vi "LinearSystemSim_Update.vi"(6 "dT_Seconds":dbl=0.02, 11 "in LinearSystemSim":T1) -> (0 "Error":bool, 3 "out LinearSystemSim":T1)   [LabVIEW 2019, in "Trajectory_Library.lvlib"]
doc: "Updates the simulation.\n \nInputs:\n - LinearSystemSim -- Data cluster\n - dtSeconds -- The time between updates.\n\nOutputs:\n - OutLinearSystemSim -- Updated data cluster\n - Error -- If TRUE, an error occured."
uses:
  Trajectory_Library.lvlib
  TypeDef/LINEAR_SYSTEM_SIM.ctl
  TypeDef/LINEAR_SYSTEM.ctl
  <vilib>/Analysis/Matrix/Datatypes/RealMatrix.ctl
  <vilib>/Analysis/Matrix/NI_Matrix.lvlib
panel:
  # "<States, 1>"
  # "<Outputs, 1>"
  # "<Inputs, 1>"
  # "<Outputs, 1>"
  # "<States,States>"
  # "<States,Inputs>"
  # "<Outputs,States>"
  # "<Outputs,Inputs>"
  # "<States, 1>"
  # "<Outputs, 1>"
  # "<Inputs, 1>"
  # "<Outputs, 1>"
  # "<States,States>"
  # "<States,Inputs>"
  # "<Outputs,States>"
  # "<Outputs,Inputs>"
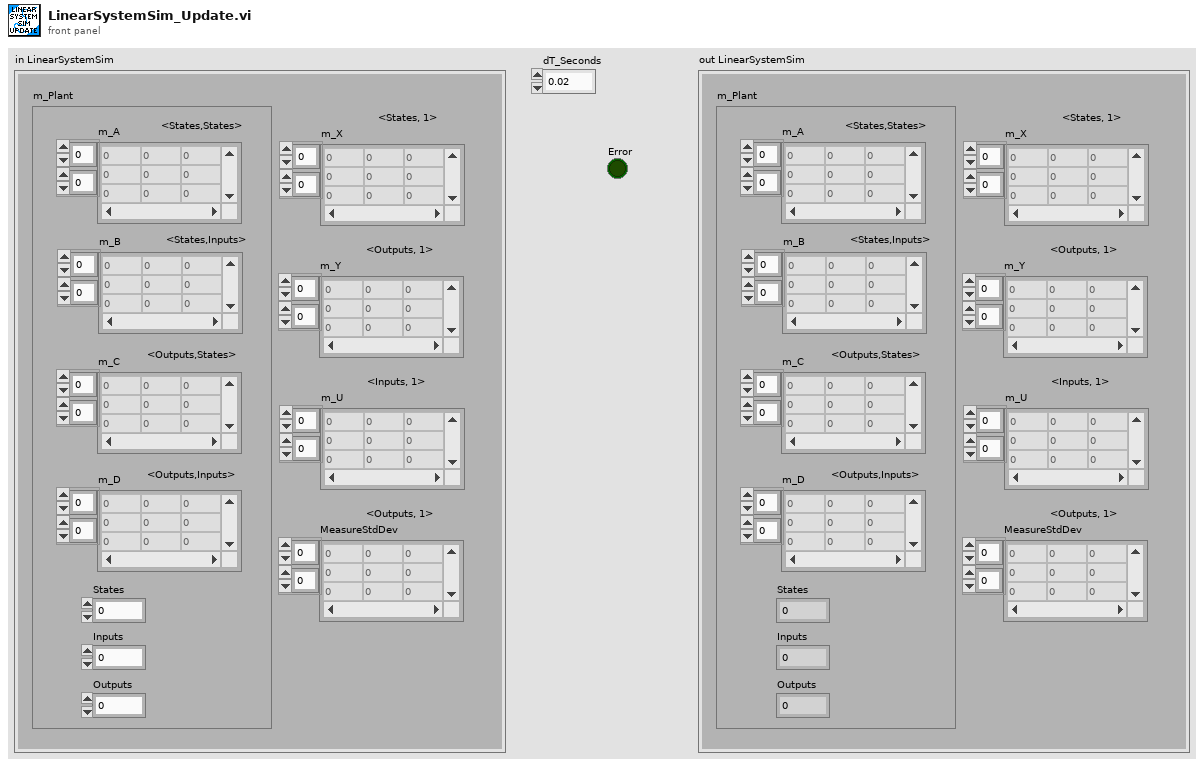
[diagram p1: front panel]
types:
  T1 = typedef "Trajectory_Library.lvlib/LINEAR_SYSTEM_SIM.ctl" = cluster{"m_Plant":T2, "m_X":T3, "m_Y":T3, "m_U":T3, "MeasureStdDev":T3}
  T2 = typedef "Trajectory_Library.lvlib/LINEAR_SYSTEM.ctl" = cluster{"m_A":T3, "m_B":T3, "m_C":T3, "m_D":T3, "States":i32, "Inputs":i32, "Outputs":i32}
  T3 = typedef "NI_Matrix.lvlib/RealMatrix.ctl" = dbl[][]
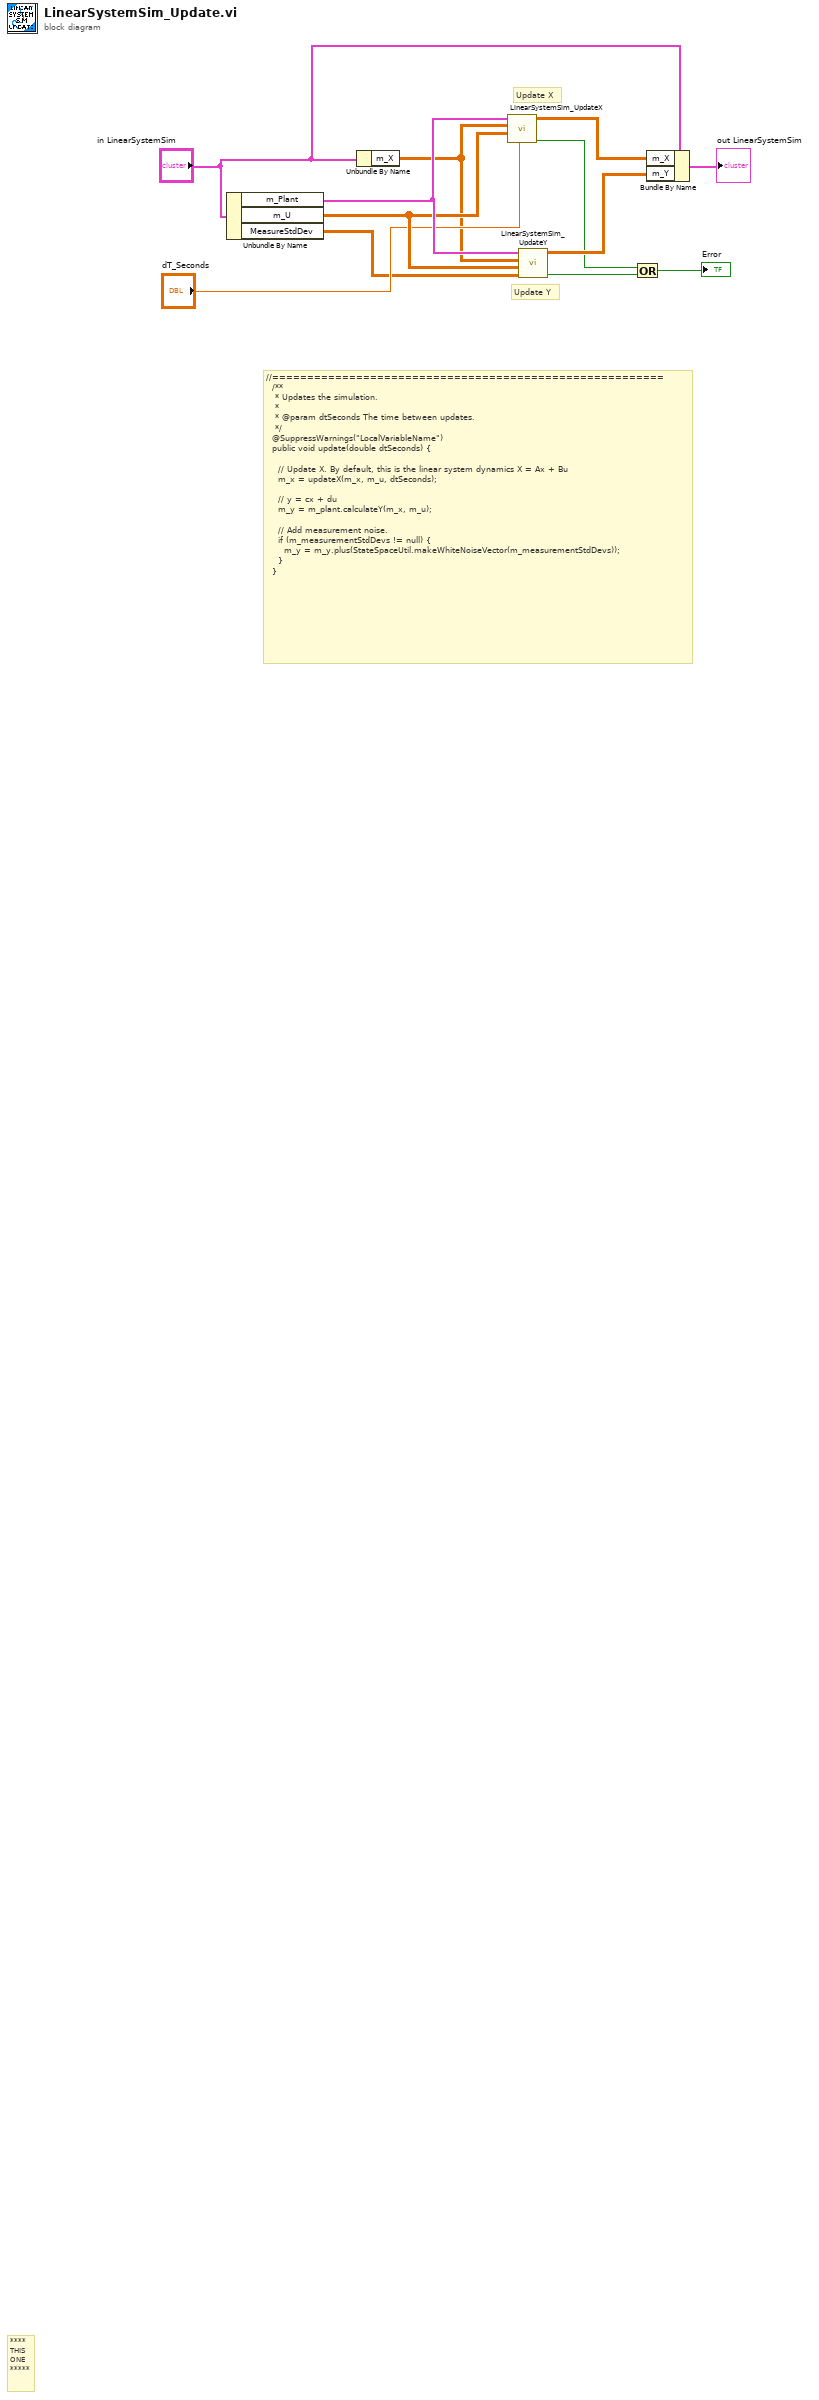
[diagram p0: block diagram]
diagram:
  # "Update Y"
  # "Update X"
  # "//========================================================\n  /**\n   * Updates the simulation.\n   *\n   * @param dtSeconds The time between updates.\n   */\n  @SuppressWarnings(\"LocalVariableName\")\n  public void update(double dtSeconds) {\n\n    // Update X. By default, this is the linear system dynamics X = Ax + Bu\n    m_x = updateX(m_x, m_u, dtSeconds);\n\n    // y = cx + du\n    m_y = m_plant.calculateY(m_x, m_u);\n\n    // Add measurement noise.\n    if (m_measurementStdDevs != null) {\n      m_y = m_y.plus(StateSpaceUtil.makeWhiteNoiseVector(m_measurementStdDevs));\n    }\n  }"
  # "****\nTHIS\nONE\n*****"
  n1 = Unbundle By Name("in LinearSystemSim") -> ("m_Plant"=w12:T2, "m_U"=w11:T3, "MeasureStdDev"=w7:T3)
  n2 = Unbundle By Name("in LinearSystemSim") -> ("m_X"=w4:T3)
  n3 = call "LinearSystemSim_UpdateX.vi"("dT_Seconds"="dT_Seconds", "U"=w11, "CurrentXHat"=w4, "in LinearSystem"=w12) -> ("Error"=w2:bool, "X"=w5:T3)  [unwired: 6 in]
  n4 = call "LinearSystemSim_UpdateY.vi"("MeasurementStdDev"=w7, "ClampedU"=w11, "X"=w4, "Linearsystem"=w12) -> ("Error"=w1:bool, "Y"=w3:T3)  [unwired: 6 in]
  n5 = Or(x=w2, y=w1) -> (x .or. y?=→"Error":bool)
  n6 = Bundle By Name(cluster="in LinearSystemSim", "m_X"=w5, "m_Y"=w3) -> (→"out LinearSystemSim":T1)
